vi "Test Server Idle is not an Error.vi"(8 "error in (no error)":errorcluster) -> (0 "error out":errorcluster)   [LabVIEW 2019, in "RemoteControl.ZMQ.Tests.lvclass"]
uses:
  RemoteControl.ZMQ.Tests.lvclass
  <vilib>/addons/_JKI Toolkits/Caraya/classes/Assert/Assert Not Error.vi
  <vilib>/addons/_JKI Toolkits/Caraya/classes/Assert/Assert True.vi
  <vilib>/addons/_JKI Toolkits/Caraya/classes/Assert/Assert.lvclass
  <vilib>/addons/_JKI Toolkits/Caraya/classes/Test/Test.lvclass
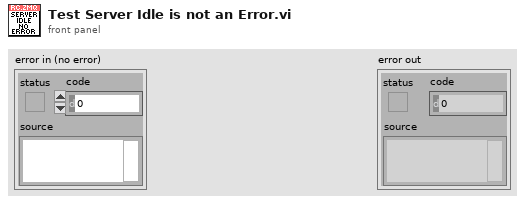
[diagram p1: front panel]
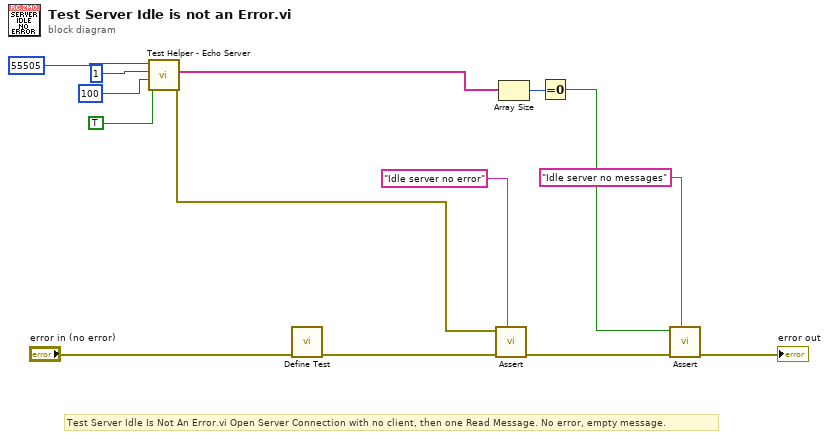
[diagram p0: block diagram]
diagram:
  # "Test Server Idle Is Not An Error.vi\tOpen Server Connection with no client, then one Read Message.\tNo error, empty message."
  n1 = call "Test Helper - Echo Server.vi"("Answer?"=TRUE, "reply delay (ms)"=u32 100, "number of messages"=1, "port"=u16 55505 ("Port")) -> ("error out"=w7:errorcluster, "Commands"=w6:string[])  [unwired: 6 in]
  n2 = call <vilib>:"Define Test.vi"("error in (no error)"="error in (no error)") -> ("error out"=w12:errorcluster)  [unwired: 9 in, 1 out]
  n3 = call-poly <vilib>:"Assert.vi"("Label"="Idle server no error", "error in (no error)"=w12, "Not Error?"=w7) -> ("error out"=w3:errorcluster)  [unwired: 7 in, 1 out]
  n4 = Array Size(array=w6) -> (size(s)=w5:i32)
  n5 = Equal To 0?(x=w5) -> (x = 0?=w4:bool)
  n6 = call-poly <vilib>:"Assert.vi"("Label"="Idle server no messages", "error in (no error)"=w3, "True?"=w4) -> ("error out"=→"error out":errorcluster)  [unwired: 7 in, 1 out]
